vi "NS_ReadWriteAttribute.vi"(0 "object in":refnum<class "NativeSubTemplate.lvclass">, 5 "Error In":errorcluster) -> (14 "object out":refnum<class "NativeSubTemplate.lvclass">, 19 "Error Out":errorcluster)   [LabVIEW 2020, in "NativeSubTemplate.lvclass"]
uses:
  NativeSubTemplate.lvclass
  NativeSubTemplate.lvclass/NativeSubTemplate.ctl
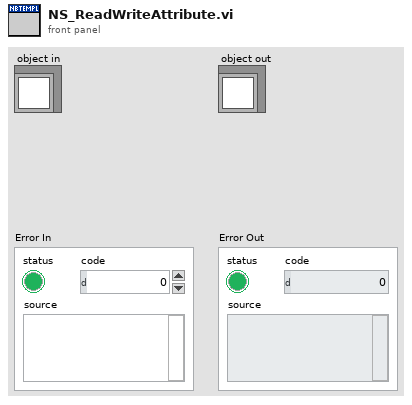
[diagram p1: front panel]
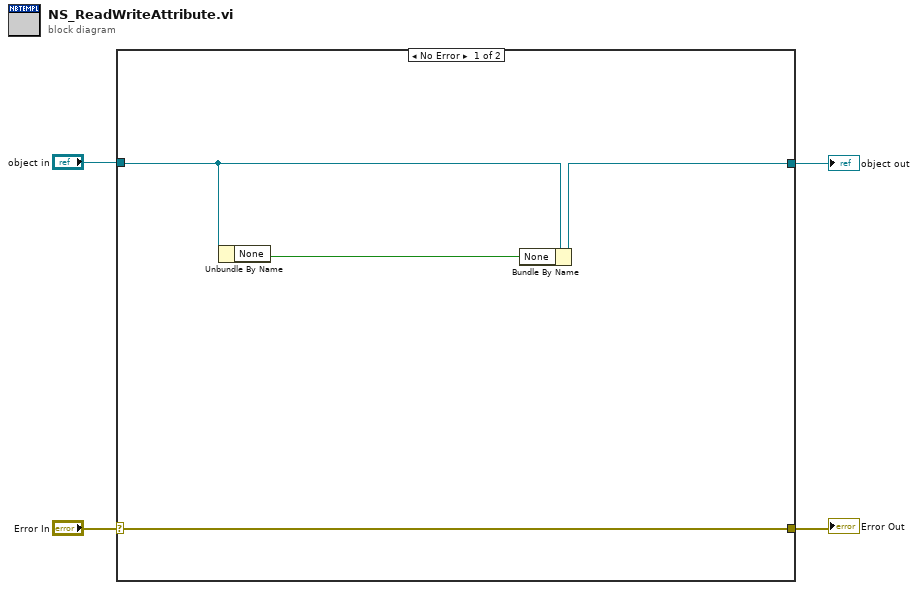
[diagram p0: block diagram]
diagram:
  n1 = case shown="No Error" "Error In" {
    selector: "Error In" -> [w7 w10]
    tunnel: [w7 w10] -> w3
    tunnel: [w5 w9] -> w1
    tunnel: "object in" -> [w6 w9]
    frame No Error {
      n2 = Unbundle By Name(w6) -> ("None"=w8:bool)
      n3 = Bundle By Name(cluster=w6, "None"=w8) -> (w5:refnum<class "NativeSubTemplate.lvclass">)
    }
    frame Error {
    }
  }
  "Error Out" <- w3
  "object out" <- w1
